vi "update Serial Port and Protocol Info.vi"(8 "error in (no error)":errorcluster, 11 "3D Controller in":refnum<class "3D Controller.lvclass">) -> (0 "error out":errorcluster, 3 "3D Controller out":refnum<class "3D Controller.lvclass">)   [LabVIEW 2023, in "FCC 3D Controller for BS.lvlib" / "3D Controller.lvclass"]
uses:
  3D Controller.lvclass
  3D Controller.lvclass/3D Controller.ctl
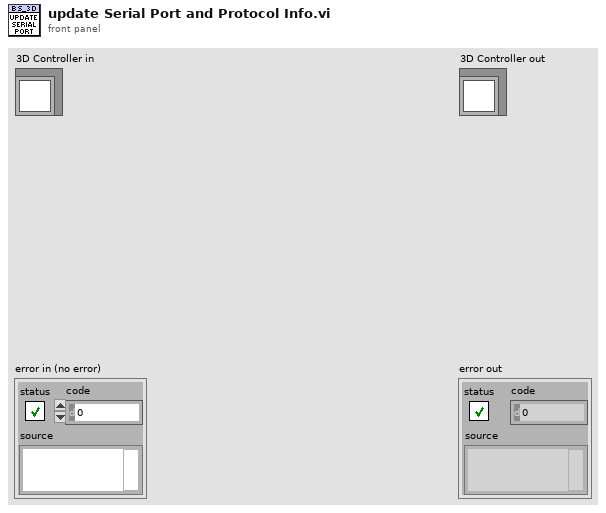
[diagram p1: front panel]
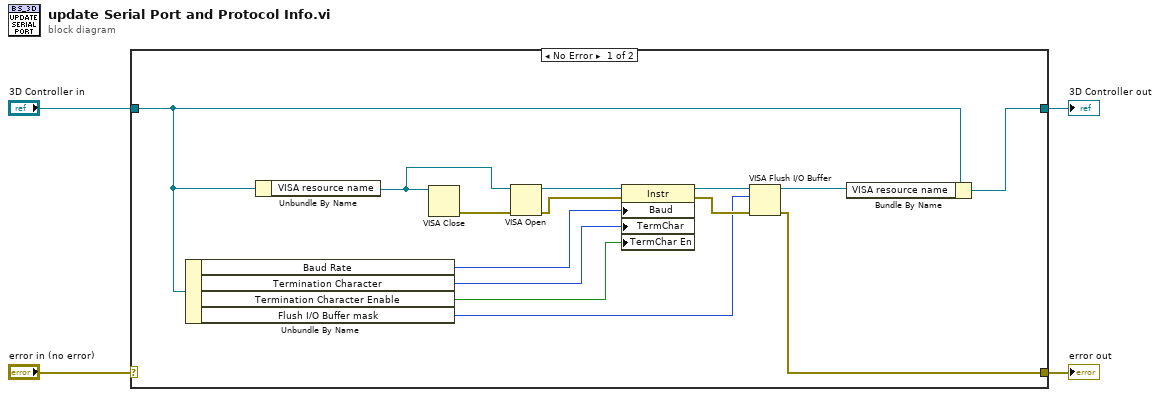
[diagram p0: block diagram]
diagram:
  n1 = case shown="No Error" "error in (no error)" {
    selector: "error in (no error)" -> [_ w20]
    tunnel: [w8 w20] -> w3
    tunnel: [w5 w19] -> w1
    tunnel: "3D Controller in" -> [w7 w19]
    frame No Error {
      n2 = Unbundle By Name(w7) -> ("Baud Rate"=w15:u32, "Termination Character"=w13:u8, "Termination Character Enable"=w12:bool, "Flush I/O Buffer mask"=w9:u16)
      n3 = Unbundle By Name(w7) -> ("VISA resource name"=w17:refnum<visa-resource-name>)
      n4 = VISA Close(VISA resource name=w17) -> (error out=w18:errorcluster)  [unwired: 1 in]
      n5 = VISA Open(error in (no error)=w18, VISA resource name=w17) -> (VISA resource name=w16:refnum<visa-resource-name>, error out=w14:errorcluster)  [unwired: 3 in]
      n6 = property class="Instr"(reference=w16, error in=w14, "Baud"=w15, "TermChar"=w13, "TermChar En"=w12) -> (reference out=w11:refnum<visa-resource-name>, error out=w10:errorcluster)
      n7 = VISA Flush I/O Buffer(VISA resource name=w11, mask (16)=w9, error in (no error)=w10) -> (VISA resource name out=w6:refnum<visa-resource-name>, error out=w8:errorcluster)
      n8 = Bundle By Name(cluster=w7, "VISA resource name"=w6) -> (w5:refnum<class "3D Controller.lvclass">)
    }
    frame Error {
    }
  }
  "error out" <- w3
  "3D Controller out" <- w1
